vi "test - String with Keywords.vi"(8 "error in (no error)":errorcluster, 11 "TestCase in":refnum<class "testcase-Supported-Datatype.lvclass">) -> (0 "error out":errorcluster, 3 "TestCase out":refnum<class "testcase-Supported-Datatype.lvclass">)   [LabVIEW 2017, in "testcase-Supported-Datatype.lvclass"]
uses:
  testcase-Supported-Datatype.lvclass
  05e71187-3928-45d8-801f-9346c6da1d9d.vi
  374b6560-8f96-4fca-b7a0-b2ea38b4c975.vi
  b40cf643-f38a-46f9-a5a3-634c21c9432c.vi
  9f15237e-ebd8-4d7f-a756-ec2da678f0ff.vi
  00d33017-f56b-420e-b77c-1e7c4d83746c.vi
  08aaf221-0d2d-4d3d-9c04-42c4c1c9dd4f.vi
  af7b55ab-96f5-4dfe-9a6e-dcc75dd624d1.vi
  addons/API-String-Arugments-Support/_Support/Convert API String Arguments to Data(variant).vi
  addons/API-String-Arugments-Support/_Support/Data To API String Arguments.vi
  <vilib>/addons/_JKI Toolkits/VI Tester/TestCase.llb/TestCase.lvclass
  C:/Program Files (x86)/National Instruments/LabVIEW 2017/vi.lib/addons/_JKI Toolkits/VI Tester/TestCase.llb/TestCase.lvclass
panel:
  out "Data":cluster{"cmd":string}
  out "API String":string
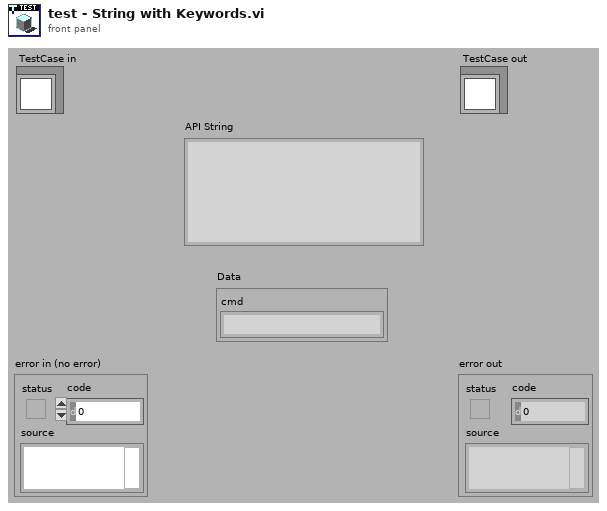
[diagram p1: front panel]
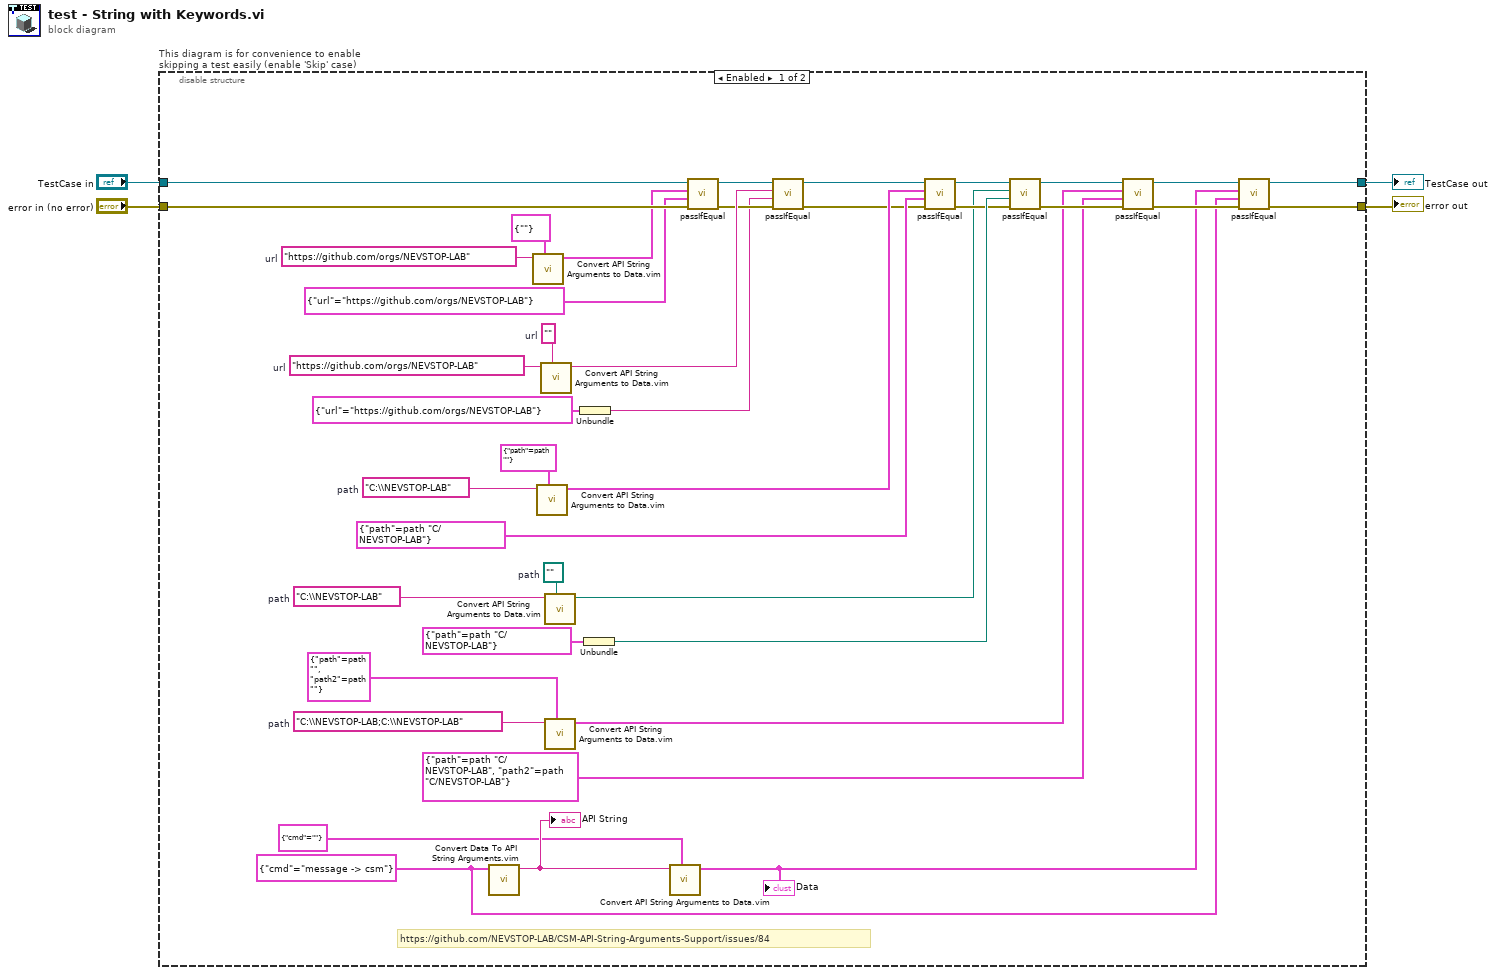
[diagram p0: block diagram]
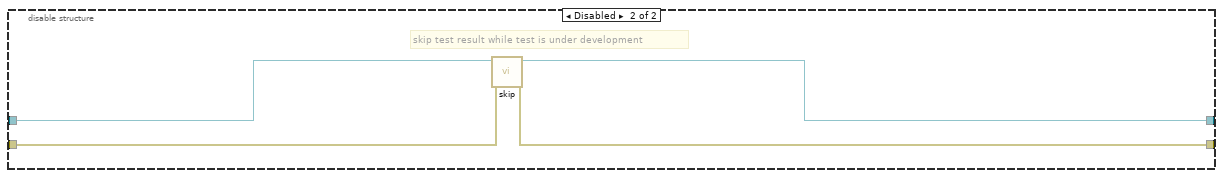
[diagram p2: hidden frame]
diagram:
  n1 = disable-structure "This diagram is for convenience to enable skipping a test easily (enable 'Skip' case)" shown="Enabled" {
    disable-tunnel: "TestCase in" -> [w44 w48]
    disable-tunnel: [w10 w46] -> w1
    disable-tunnel: [w9 w47] -> w3
    disable-tunnel: "error in (no error)" -> [w43 w45]
    frame Enabled {
      w5 = cluster{"cmd":string} {"cmd"="message -> csm"}
      w18 = "C:\\NEVSTOP-LAB;C:\\NEVSTOP-LAB"  # path
      w30 = path ""  # path
      w27 = "C:\\NEVSTOP-LAB"  # path
      w22 = "C:\\NEVSTOP-LAB"  # path
      w33 = ""  # url
      w36 = "https://github.com/orgs/NEVSTOP-LAB"  # url
      w41 = "https://github.com/orgs/NEVSTOP-LAB"  # url
      # "https://github.com/NEVSTOP-LAB/CSM-API-String-Arguments-Support/issues/84"
      n2 = call "Convert Data To API String Arguments.vim"("Data"=w5) -> ("API String"=w8:string)  [unwired: 7 in, 1 out]
      "API String" <- w8
      n3 = call "Convert API String Arguments to Data.vim"("Reference Type"=cluster{"url":string} {"url"=""}, "API String"=w41) -> ("Data"=w40:cluster{"url":string})  [unwired: 6 in, 1 out]
      n4 = call "Convert API String Arguments to Data.vim"("Reference Type"=cluster{"path":path} {"path"=path ""}, "API String"=w22) -> ("Data"=w23:cluster{"path":path})  [unwired: 6 in, 1 out]
      n5 = call "Convert API String Arguments to Data.vim"("Reference Type"=w33, "API String"=w36) -> ("Data"=w37:string)  [unwired: 6 in, 1 out]
      n6 = call "Convert API String Arguments to Data.vim"("Reference Type"=w30, "API String"=w27) -> ("Data"=w26:path)  [unwired: 6 in, 1 out]
      n7 = call "Convert API String Arguments to Data.vim"("Reference Type"=cluster{"path":path, "path2":path} {"path"=path "", "path2"=path ""}, "API String"=w18) -> ("Data"=w14:cluster{"path":path, "path2":path})  [unwired: 6 in, 1 out]
      n8 = Unbundle(cluster{"url":string} {"url"="https://github.com/orgs/NEVSTOP-LAB"}) -> ("url"=w32:string)
      n9 = Unbundle(cluster{"path":path} {"path"=path "C:/NEVSTOP-LAB"}) -> ("path"=w31:path)
      n10 = call "Convert API String Arguments to Data.vim"("Reference Type"=cluster{"cmd":string} {"cmd"=""}, "API String"=w8) -> ("Data"=w6:cluster{"cmd":string})  [unwired: 6 in, 1 out]
      "Data" <- w6
      n11 = call-dynamic "passIfEqual.vi"("error in (no error)"=w43, "y"=cluster{"url":string} {"url"="https://github.com/orgs/NEVSTOP-LAB"}, "x"=w40, "TestCase in"=w44) -> ("error out"=w34:errorcluster, "TestCase out"=w35:refnum<class "testcase-Supported-Datatype.lvclass">)  [unwired: 6 in]
      n12 = call-dynamic "passIfEqual.vi"("error in (no error)"=w34, "y"=w32, "x"=w37, "TestCase in"=w35) -> ("error out"=w19:errorcluster, "TestCase out"=w20:refnum<class "testcase-Supported-Datatype.lvclass">)  [unwired: 6 in]
      n13 = call-dynamic "passIfEqual.vi"("error in (no error)"=w19, "y"=cluster{"path":path} {"path"=path "C:/NEVSTOP-LAB"}, "x"=w23, "TestCase in"=w20) -> ("error out"=w29:errorcluster, "TestCase out"=w28:refnum<class "testcase-Supported-Datatype.lvclass">)  [unwired: 6 in]
      n14 = call-dynamic "passIfEqual.vi"("error in (no error)"=w29, "y"=w31, "x"=w26, "TestCase in"=w28) -> ("error out"=w15:errorcluster, "TestCase out"=w16:refnum<class "testcase-Supported-Datatype.lvclass">)  [unwired: 6 in]
      n15 = call-dynamic "passIfEqual.vi"("error in (no error)"=w15, "y"=cluster{"path":path, "path2":path} {"path"=path "C:/NEVSTOP-LAB", "path2"=path "C:/NEVSTOP-LAB"}, "x"=w14, "TestCase in"=w16) -> ("error out"=w12:errorcluster, "TestCase out"=w11:refnum<class "testcase-Supported-Datatype.lvclass">)  [unwired: 6 in]
      n16 = call-dynamic "passIfEqual.vi"("error in (no error)"=w12, "y"=w5, "x"=w6, "TestCase in"=w11) -> ("error out"=w9:errorcluster, "TestCase out"=w10:refnum<class "testcase-Supported-Datatype.lvclass">)  [unwired: 6 in]
    }
    frame Disabled {
      # "skip test result while test is under development"
      n17 = call <vilib>:"skip.vi"("error in (no error)"=w45, "TestCase in"=w48) -> ("error out"=w47:errorcluster, "TestCase out"=w46:refnum<class "testcase-Supported-Datatype.lvclass">)  [unwired: 8 in]
    }
  }
  "error out" <- w3
  "TestCase out" <- w1
